vi "mythirdlabview.vi"() -> ()   [LabVIEW 2026]
uses:
  <vilib>/picture/picture.llb/imagedata.ctl
panel:
  out "grid error":bool
  out "# cols":i32
  out "#rows":i32
  out "error out 2":errorcluster
  in  "error in":errorcluster
  out "error out":errorcluster
  out "Cell values":string
  out "standard error":string
  out "standard output":string
  out "text":string
  in  "Path":path
  out "stripped sub path":path
  out "name 2":string
  out "stripped path":path
  out "name":string
  out "1-bit cell image":bool[][](array[boolean])
  out "cell":picture
  out "row 10":bool[](array[boolean])
  out "B&W picture":picture
  out "image data":T1
  out "px":bool[](array[boolean])
  out "1-bit pixmap":bool[][](array[boolean])
  out "color Picture":picture
  in  "PNG Path":path
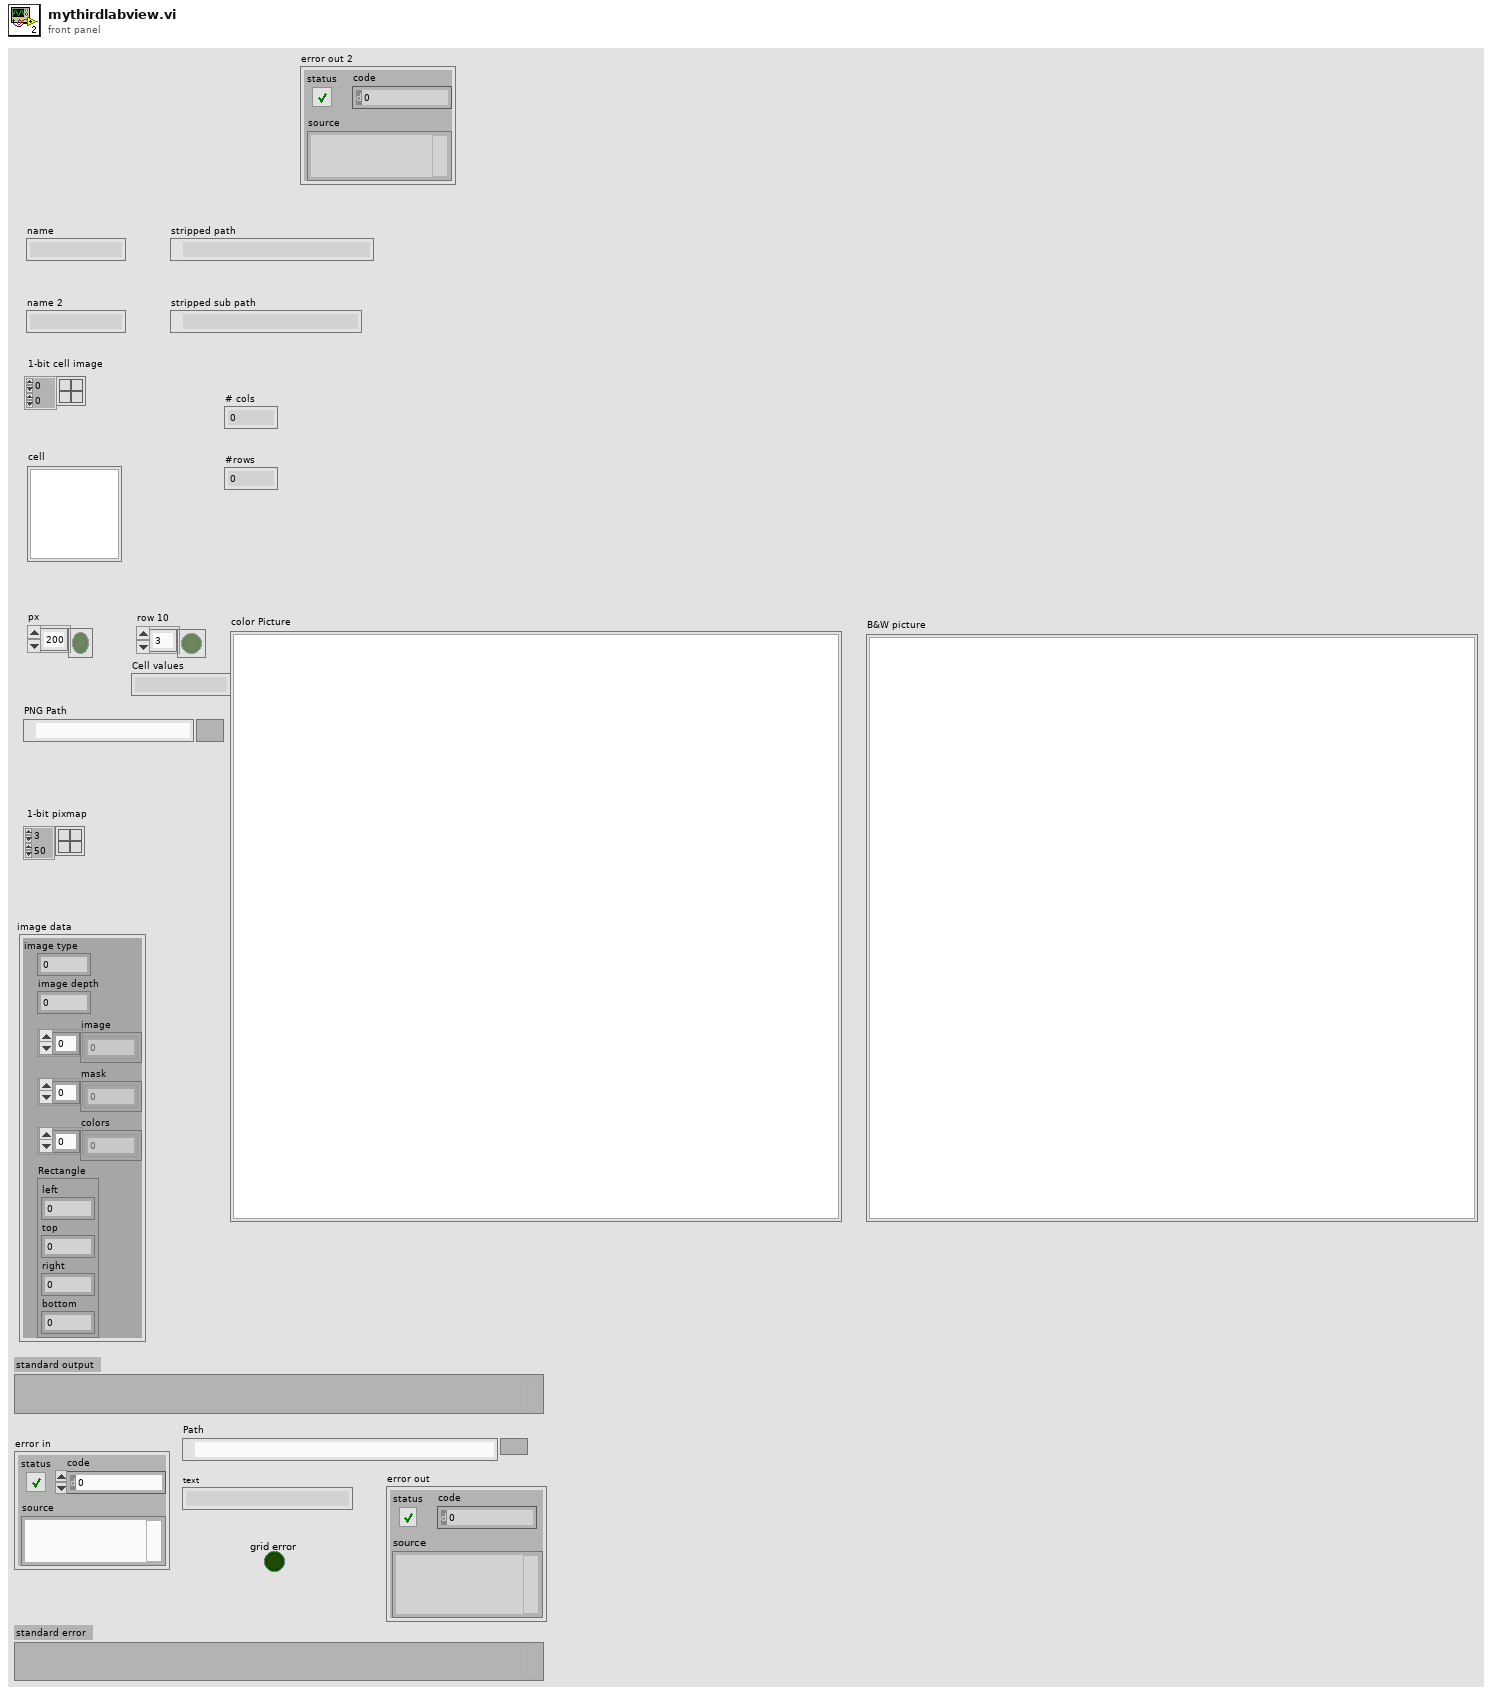
[diagram p1: front panel]
types:
  T1 = typedef "imagedata.ctl" = cluster{"image type":i32, "image depth":i32, "image":u8[], "mask":u8[], "colors":u32[], "Rectangle":cluster{"left":i16, "top":i16, "right":i16, "bottom":i16}}
  T2 = enum16{"big-endian, network order", "native, host order", "little-endian"}
  T3 = cluster{"left":i16, "top":i16, "right":i16, "bottom":i16}
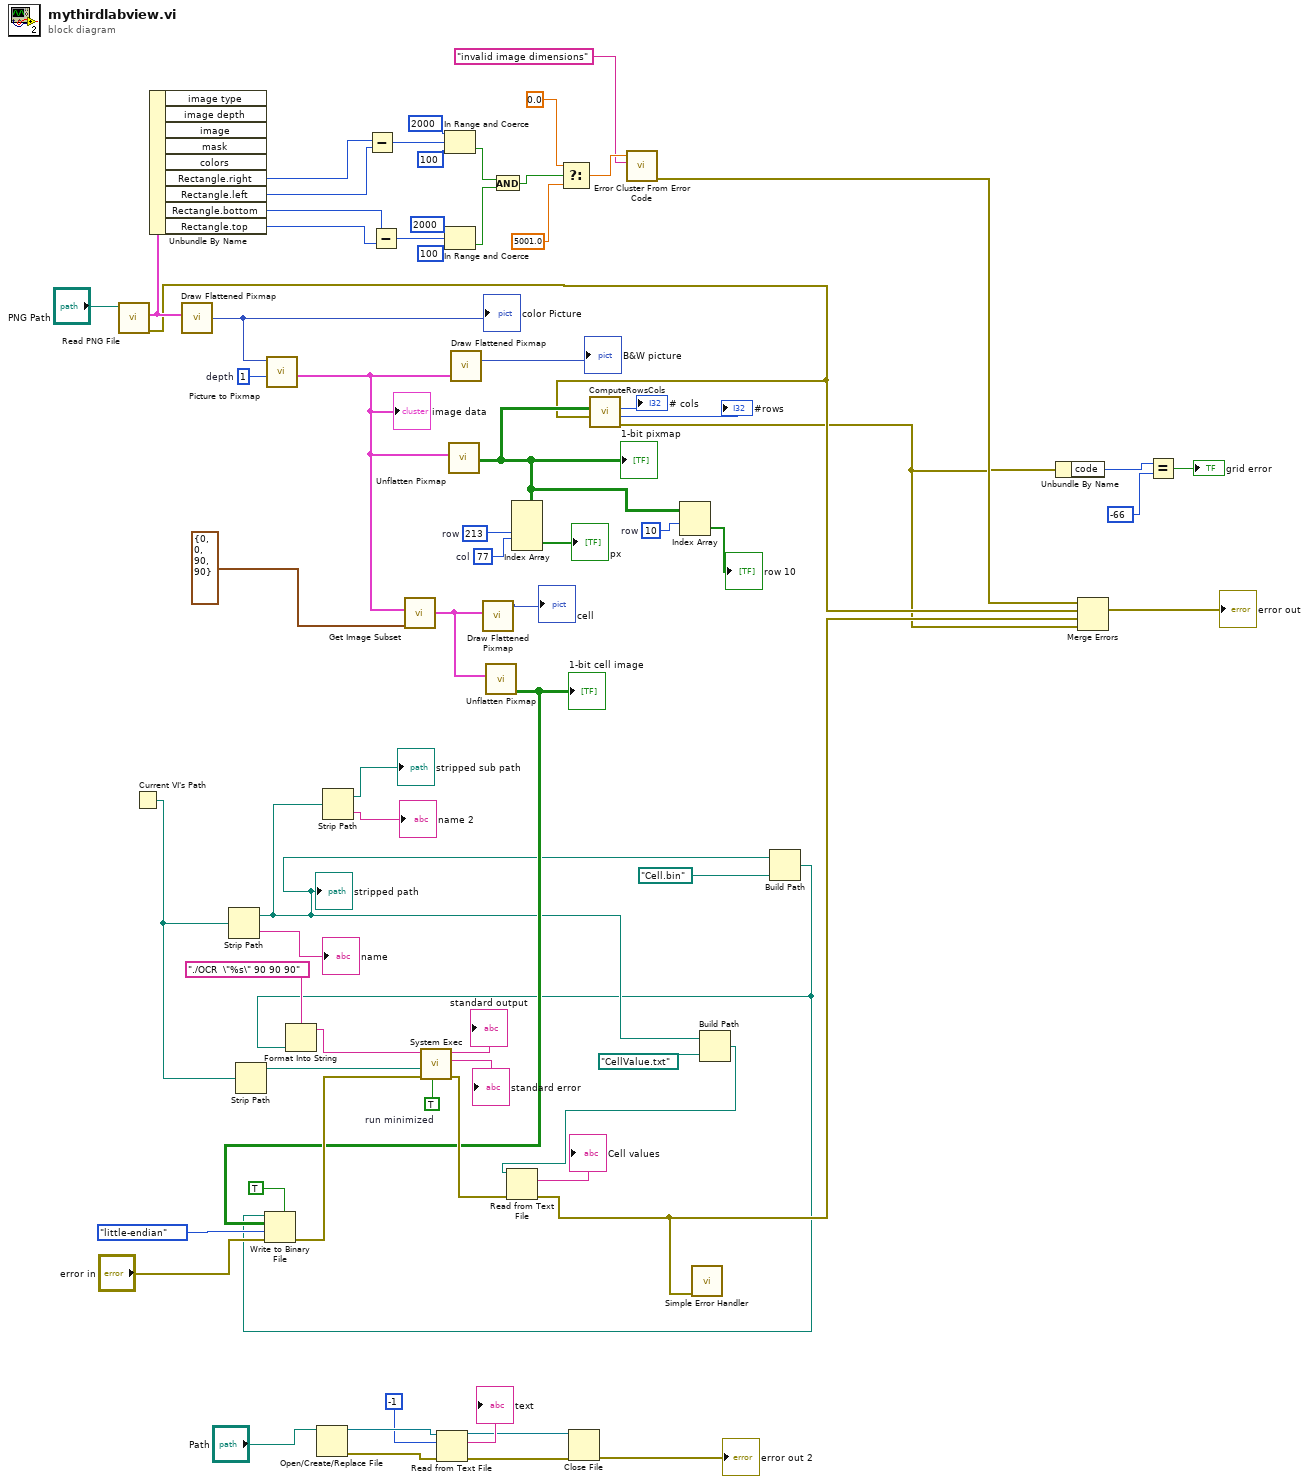
[diagram p0: block diagram]
diagram:
  w47 = TRUE  # run minimized
  w65 = 10  # row
  w68 = 77  # col
  w69 = 213  # row
  w70 = 1  # depth
  n1 = call <vilib>:"Read PNG File.vi"("path to PNG file"="PNG Path") -> ("error out"=w7:errorcluster, "image data"=w60:T1)  [unwired: 8 in, 1 out]
  n2 = Current VI's Path() -> (path=w51:path)
  n3 = Unbundle By Name(w60) -> ("Rectangle.right"=w21:i16, "Rectangle.left"=w22:i16, "Rectangle.bottom"=w24:i16, "Rectangle.top"=w23:i16)  [unwired: 5 out]
  n4 = call <vilib>:"Draw Flattened Pixmap.vi"("image data"=w60) -> ("new picture"=w71:picture)  [unwired: 8 in]
  "color Picture" <- w71
  n5 = Strip Path(path=w51) -> (stripped path=w12:path, name=→"name":string)
  "stripped path" <- w12
  n6 = Strip Path(path=w51) -> (stripped path=w50:path)  [unwired: 1 out]
  n7 = call <vilib>:"Picture to Pixmap.vi"("depth"=w70, "picture"=w71) -> ("image data"=w63:T1)  [unwired: 8 in, 1 out]
  "image data" <- w63
  n8 = Open/Create/Replace File(file path (use dialog)="Path") -> (refnum out=w55:refnum<file>, error out=w46:errorcluster)  [unwired: 5 in, 1 out]
  n9 = Strip Path(path=w12) -> (stripped path=→"stripped sub path":path, name=→"name 2":string)
  n10 = Subtract(x=w21, y=w22) -> (x-y=w37:i16)
  n11 = Subtract(x=w24, y=w23) -> (x-y=w36:i16)
  n12 = call <vilib>:"Get Image Subset.vi"("subset rect"=T3 {"left"=0, "top"=0, "right"=90, "bottom"=90}, "image data"=w63) -> ("image subset"=w62:T1)  [unwired: 4 in, 1 out]
  n13 = Read from Text File(file (use dialog)=w55, count=-1, error in=w46) -> (refnum out=w52:refnum<file>, text=→"text":string, error out=w45:errorcluster)  [unwired: 1 in, 1 out]
  n14 = In Range and Coerce(upper limit=i16 2000, x=w37, lower limit=i16 100) -> (In Range?=w31:bool)  [unwired: 1 out]
  n15 = In Range and Coerce(upper limit=i16 2000, x=w36, lower limit=i16 100) -> (In Range?=w30:bool)  [unwired: 1 out]
  n16 = call <vilib>:"Unflatten Pixmap.vi"("image data"=w63) -> ("1-bit pixmap"=w8:bool[][])  [unwired: 4 in, 6 out]
  "1-bit pixmap" <- w8
  n17 = call <vilib>:"Draw Flattened Pixmap.vi"("image data"=w63) -> ("new picture"=→"B&W picture":picture)  [unwired: 8 in]
  n18 = call <vilib>:"Draw Flattened Pixmap.vi"("image data"=w62) -> ("new picture"=→"cell":picture)  [unwired: 8 in]
  n19 = call <vilib>:"Unflatten Pixmap.vi"("image data"=w62) -> ("1-bit pixmap"=w38:bool[][])  [unwired: 4 in, 6 out]
  "1-bit cell image" <- w38
  n20 = And(x=w31, y=w30) -> (x .and. y?=w28:bool)
  n21 = Index Array(array=w8, index (row) #1=w69, index (row) #2=w68) -> (element #2=→"px":bool[])  [unwired: 2 in, 1 out]
  n22 = Select(t=0.0, s=w28, f=5001.0) -> (s? t:f=w26:dbl)
  n23 = Close File(refnum=w52, error in=w45) -> (error out=→"error out 2":errorcluster)  [unwired: 1 out]
  n24 = call "ComputeRowsCols.vi"("error in (no error)"=w7, "1-bit pixmap"=w8) -> ("error out"=w4:errorcluster, "#rows"=→"#rows":i32, "# cols"=→"# cols":i32)  [unwired: 7 in]
  n25 = call <vilib>:"Error Cluster From Error Code.vi"("error message (\"\")"="invalid image dimensions", "error code (0)"=w26) -> ("error out"=w19:errorcluster)  [unwired: 7 in]
  n26 = Index Array(array=w8, index (row)=w65) -> (element=→"row 10":bool[])  [unwired: 1 in]
  n27 = Build Path(base path=w12, name or relative path=path "CellValue.txt") -> (appended path=w10:path)
  n28 = Build Path(base path=w12, name or relative path=path "Cell.bin") -> (appended path=w9:path)
  n29 = Write to Binary File(file (use dialog)=w9, data=w38, error in="error in", 5:TRUE ("prepend array or string size? (T)"), 9:T2."little-endian" ("byte order (0:big-endian, network order)")) -> (error out=w44:errorcluster)  [unwired: 1 in, 2 out]
  n30 = Format Into String(format string="./OCR  \"%s\" 90 90 90" ("standard input"), w9) -> (resulting string=w15:string)  [unwired: 2 in, 1 out]
  n31 = call <vilib>:"System Exec.vi"("run minimized? (F)"=w47, "error in (no error)"=w44, "working directory"=w50, "command line"=w15) -> ("error out"=w43:errorcluster, "standard error"=→"standard error":string, "standard output"=→"standard output":string)  [unwired: 4 in, 1 out]
  n32 = Read from Text File(file (use dialog)=w10, error in=w43) -> (text=→"Cell values":string, error out=w18:errorcluster)  [unwired: 2 in, 2 out]
  n33 = call <vilib>:"Simple Error Handler.vi"("error in (no error)"=w18) -> ()  [unwired: 4 in, 5 out]
  n34 = Unbundle By Name(w4) -> ("code"=w3:i32)
  n35 = Merge Errors(w19, w7, w18, w4) -> (→"error out":errorcluster)
  n36 = Equal?(x=w3, y=-66) -> (x = y?=→"grid error":bool)
